vi "[ce] ODE Solver - Prepare expression.vi"(4 "method":enum16{"Runge Kutta", "Euler"}(ring), 6 "equation parameters":T1(array[cluster]) {"x0" format="%.2f"}, 8 "error in":errorcluster, 9 "variable names":T2(array[cluster]), 10 "time names":T3) -> (0 "error out":errorcluster, 3 "expression":string)   [LabVIEW 2021]
doc: "::: CalcExpress Toolkit :::\nCopyright (c) 2000-2026 Konstantin Shifershteyn. All rights reserved."
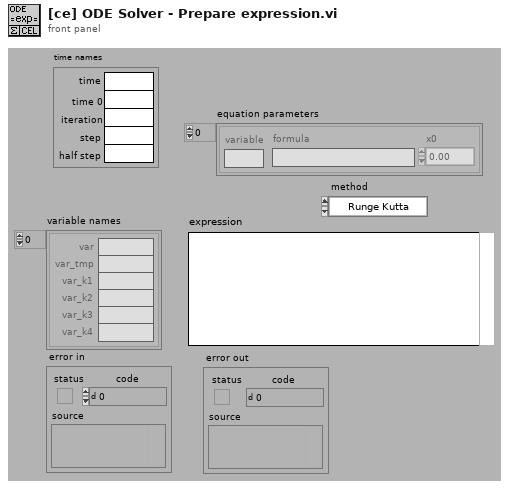
[diagram p1: front panel]
types:
  T1 = cluster{"variable":string, "formula":string, "x0":dbl}[]
  T2 = cluster{"var":string, "var_tmp":string, "var_k1":string, "var_k2":string, "var_k3":string, "var_k4":string}[]
  T3 = cluster{"time":string, "time 0":string, "iteration":string, "step":string, "half step":string}
  T4 = cluster{"variable":string, "formula":string, "x0":dbl}
  T5 = cluster{"var":string, "var_tmp":string, "var_k1":string, "var_k2":string, "var_k3":string, "var_k4":string}
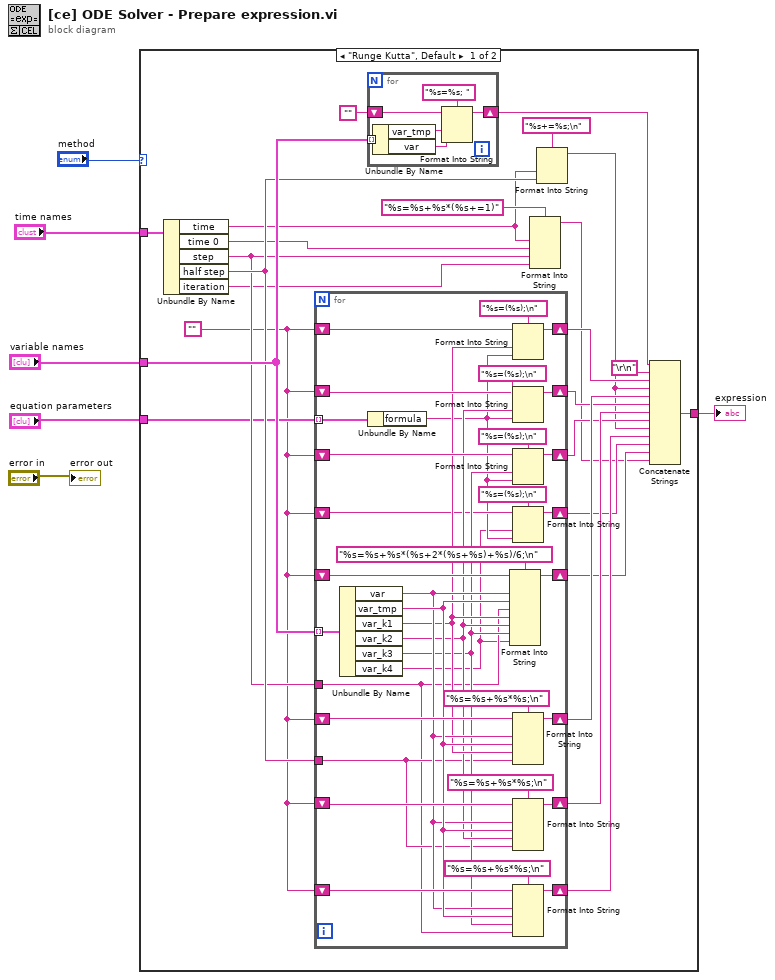
[diagram p0: block diagram]
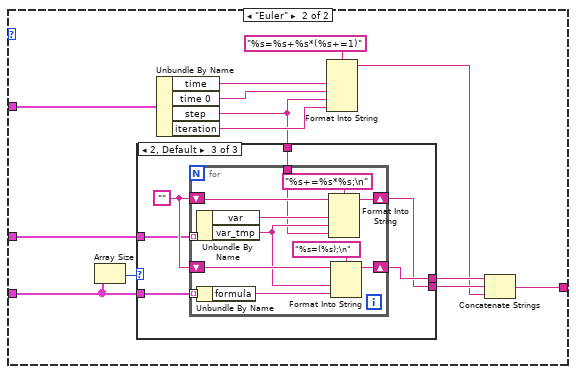
[diagram p2: hidden frame]
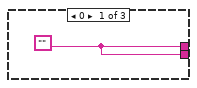
[diagram p3: hidden frame]
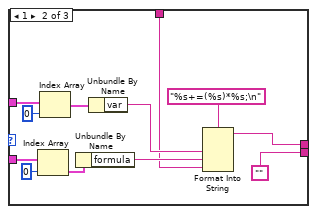
[diagram p4: hidden frame]
diagram:
  n1 = case shown="\"Runge Kutta\", Default" "method" {
    tunnel: "time names" -> [w31 w82]
    tunnel: "variable names" -> [w30 w83]
    tunnel: [w17 w81] -> w1
    tunnel: "equation parameters" -> [w16 w73]
    frame "Runge Kutta", Default {
      w15 = "" ("Empty String Constant")
      n2 = Unbundle By Name(w31) -> ("time"=w9:string, "time 0"=w11:string, "step"=w26:string, "half step"=w27:string, "iteration"=w12:string)
      n3 = for {
        shift-right: [w65] -> w23
        shift-left: w15 -> [w66]
        tunnel: w16 -> [w61] mode=indexing
        tunnel: w26 -> [w38]
        shift-right: [w60] -> w13
        shift-left: w15 -> [w58]
        shift-right: [w59] -> w19
        shift-left: w15 -> [w57]
        shift-right: [w56] -> w21
        shift-left: w15 -> [w55]
        tunnel: w30 -> [w54] mode=indexing
        tunnel: w27 -> [w39]
        shift-right: [w50] -> w22
        shift-left: w15 -> [w49]
        shift-right: [w47] -> w20
        shift-left: w15 -> [w48]
        shift-right: [w46] -> w18
        shift-left: w15 -> [w45]
        shift-right: [w35] -> w14
        shift-left: w15 -> [w36]
        n4 = Unbundle By Name(w54) -> ("var"=w43:string, "var_tmp"=w44:string, "var_k1"=w42:string, "var_k2"=w41:string, "var_k3"=w40:string, "var_k4"=w33:string)
        n5 = Unbundle By Name(w61) -> ("formula"=w34:string)
        n6 = Format Into String(format string="%s=%s+%s*(%s+2*(%s+%s)+%s)/6;\n" ("Format String"), initial string=w58, w43, w44, w38, w42, w41, w40, w33) -> (resulting string=w60:string)  [unwired: 1 in, 1 out]
        n7 = Format Into String(format string="%s=(%s);\n" ("Format String"), initial string=w66, w42, w34) -> (resulting string=w65:string)  [unwired: 1 in, 1 out]
        n8 = Format Into String(format string="%s=(%s);\n" ("Format String"), initial string=w55, w41, w34) -> (resulting string=w56:string)  [unwired: 1 in, 1 out]
        n9 = Format Into String(format string="%s=(%s);\n" ("Format String"), initial string=w57, w40, w34) -> (resulting string=w59:string)  [unwired: 1 in, 1 out]
        n10 = Format Into String(format string="%s=(%s);\n" ("Format String"), initial string=w36, w33, w34) -> (resulting string=w35:string)  [unwired: 1 in, 1 out]
        n11 = Format Into String(format string="%s=%s+%s*%s;\n" ("Format String"), initial string=w49, w43, w44, w42, w39) -> (resulting string=w50:string)  [unwired: 1 in, 1 out]
        n12 = Format Into String(format string="%s=%s+%s*%s;\n" ("Format String"), initial string=w48, w43, w44, w41, w39) -> (resulting string=w47:string)  [unwired: 1 in, 1 out]
        n13 = Format Into String(format string="%s=%s+%s*%s;\n" ("Format String"), initial string=w45, w43, w44, w40, w38) -> (resulting string=w46:string)  [unwired: 1 in, 1 out]
      }
      n14 = for {
        shift-right: [w71] -> w25
        shift-left: "" ("Empty String Constant") -> [w72]
        tunnel: w30 -> [w68] mode=indexing
        n15 = Unbundle By Name(w68) -> ("var_tmp"=w70:string, "var"=w69:string)
        n16 = Format Into String(format string="%s=%s; " ("Format String"), initial string=w72, w70, w69) -> (resulting string=w71:string)  [unwired: 1 in, 1 out]
      }
      n17 = Format Into String(format string="%s=%s+%s*(%s+=1)" ("Format String"), w9, w11, w26, w12) -> (resulting string=w8:string)  [unwired: 2 in, 1 out]
      n18 = Format Into String(format string="%s+=%s;\n" ("Format String"), w9, w27) -> (resulting string=w7:string)  [unwired: 2 in, 1 out]
      n19 = Concatenate Strings(w25, "\r\n" ("End of Line Constant"), w23, w7, w22, w21, w20, w19, w7, w18, w14, w13, w8) -> (w17:string)
    }
    frame "Euler" {
      n20 = Array Size(array=w73) -> (size(s)=w74:i32)
      n21 = Unbundle By Name(w82) -> ("time"=w76:string, "time 0"=w79:string, "step"=w75:string, "iteration"=w78:string)
      n22 = case shown="2, Default" w74 {
        tunnel: [w86 w98 w104] -> w85
        tunnel: [w86 "" ("Empty String Constant") w103] -> w84
        tunnel: w73 -> [_ w96 w101]
        tunnel: w83 -> [_ w94 w100]
        tunnel: w75 -> [_ w87 w99]
        frame 0 {
          w86 = "" ("Empty String Constant")
        }
        frame 1 {
          n23 = Index Array(array=w96, index=0 ("Index")) -> (element=w95:T4)
          n24 = Index Array(array=w94, index=0 ("Index")) -> (element=w93:T5)
          n25 = Unbundle By Name(w95) -> ("formula"=w97:string)
          n26 = Unbundle By Name(w93) -> ("var"=w88:string)
          n27 = Format Into String(format string="%s+=(%s)*%s;\n", w88, w97, w87) -> (resulting string=w98:string)  [unwired: 2 in, 1 out]
        }
        frame 2, Default {
          w102 = "" ("Empty String Constant")
          n28 = for {
            shift-right: [w115] -> w104
            shift-left: w102 -> [w116]
            tunnel: w101 -> [w113] mode=indexing
            tunnel: w100 -> [w112] mode=indexing
            shift-right: [w110] -> w103
            shift-left: w102 -> [w109]
            tunnel: w99 -> [w106]
            n29 = Unbundle By Name(w112) -> ("var"=w108:string, "var_tmp"=w107:string)
            n30 = Unbundle By Name(w113) -> ("formula"=w105:string)
            n31 = Format Into String(format string="%s+=%s*%s;\n" ("Format String"), initial string=w109, w108, w107, w106) -> (resulting string=w110:string)  [unwired: 1 in, 1 out]
            n32 = Format Into String(format string="%s=(%s);\n" ("Format String"), initial string=w116, w107, w105) -> (resulting string=w115:string)  [unwired: 1 in, 1 out]
          }
        }
      }
      n33 = Format Into String(format string="%s=%s+%s*(%s+=1)" ("Format String"), w76, w79, w75, w78) -> (resulting string=w77:string)  [unwired: 2 in, 1 out]
      n34 = Concatenate Strings(w85, w84, w77) -> (w81:string)
    }
  }
  "expression" <- w1
  "error out" <- "error in"
